vi "GOOP_ProviderClasses_SortingDialog.vi"(8 "error in (no error)":errorcluster) -> (0 "error out":errorcluster, 2 "Cancelled":bool, 3 "FirstProvider":string)   [LabVIEW 2020]
panel:
  in  "Cancel":bool
  in  "Save":bool
  in  "Down":bool
  in  "Up":bool
  in  "ClassProviders":i32(listbox) caption="Class Providers Order"
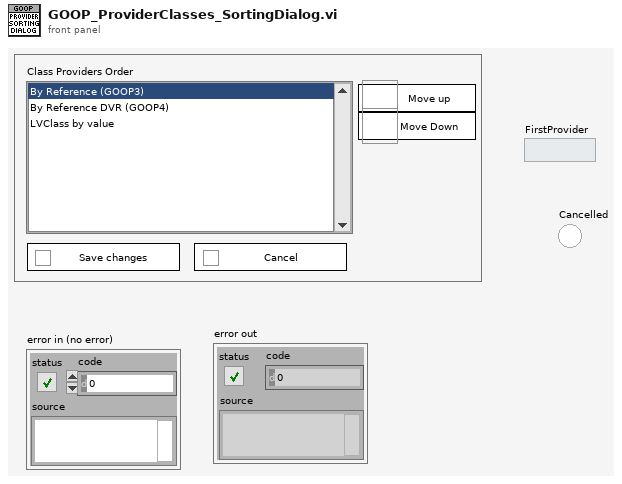
[diagram p1: front panel]
types:
  T1 = cluster{"Providers":cluster{"Provider":string, "Active":bool, "TranslatedName":string}[], "Provider":string, "Cancelled":bool}
  T2 = cluster{"Provider":string, "Active":bool, "TranslatedName":string}
  T3 = enum8{"Enabled", "Disabled", "Disabled and Grayed Out"}
  T4 = cluster{"Provider":string, "Active":bool, "TranslatedName":string}[]
  T5 = typedef "LVPoint32TypeDef.ctl" = cluster{"Horizontal":i32, "Vertical":i32}
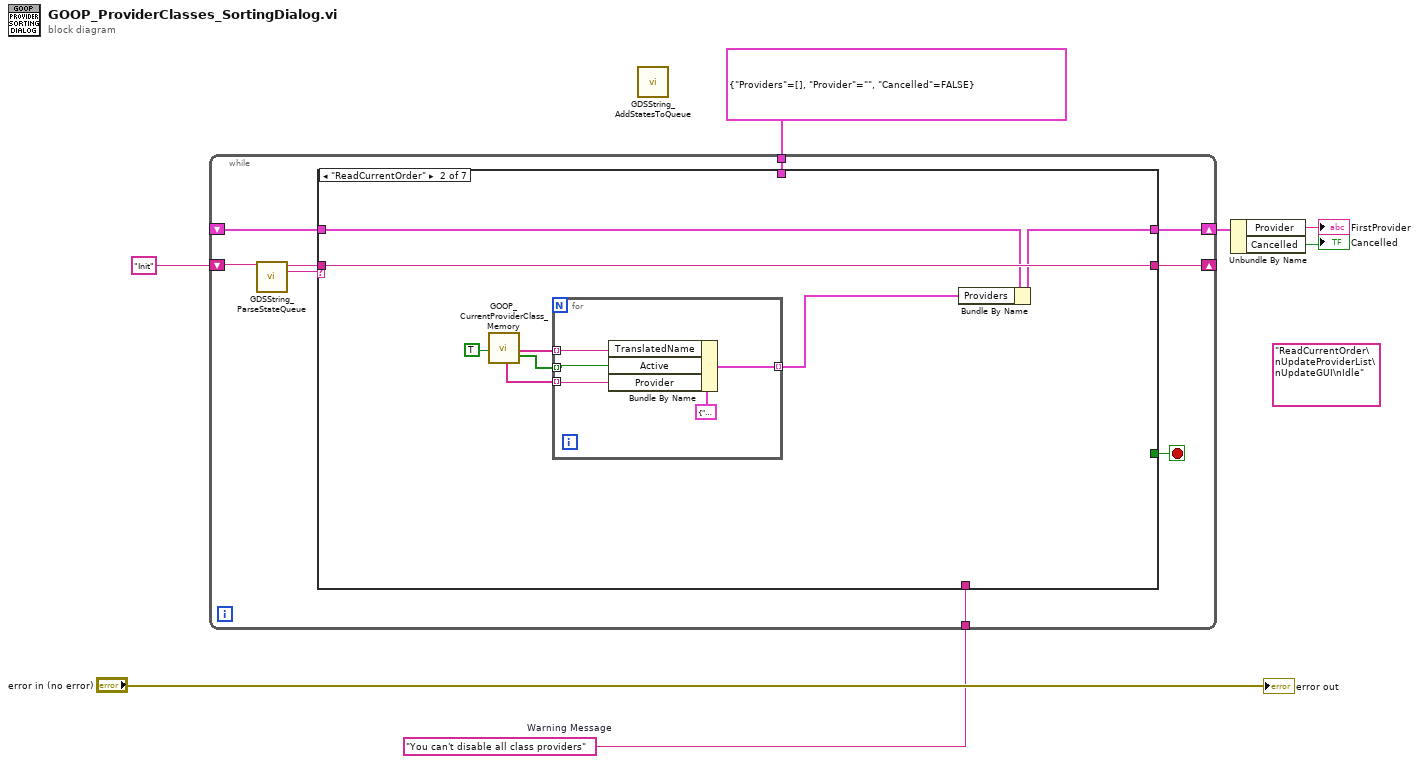
[diagram p0: block diagram]
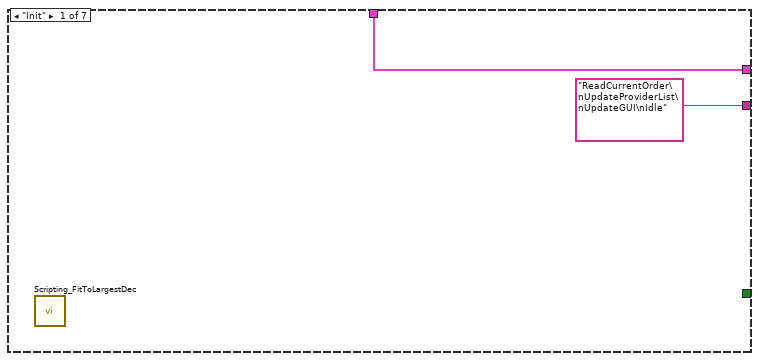
[diagram p2: hidden frame]
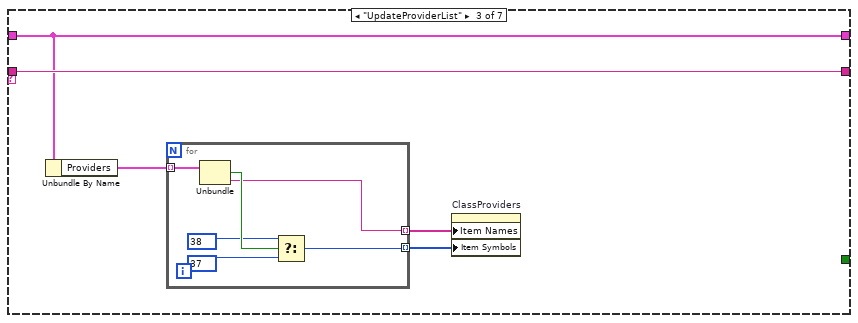
[diagram p3: hidden frame]
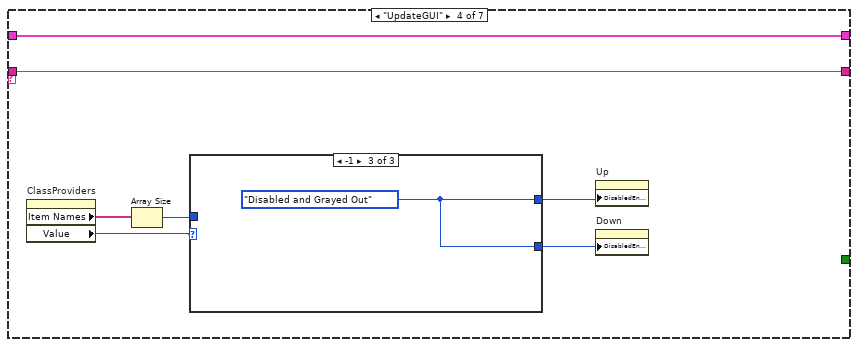
[diagram p4: hidden frame]
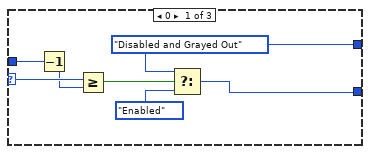
[diagram p5: hidden frame]
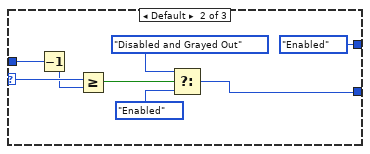
[diagram p6: hidden frame]
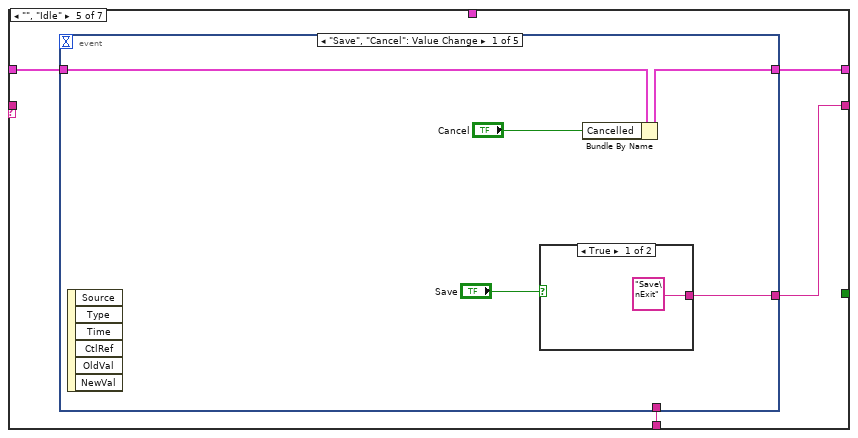
[diagram p7: hidden frame]
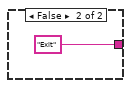
[diagram p8: hidden frame]
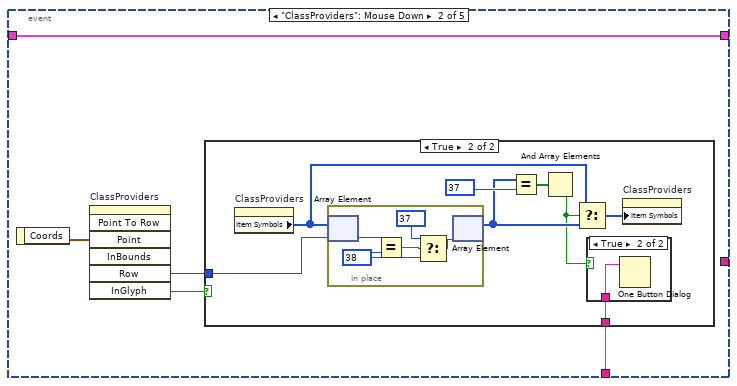
[diagram p9: hidden frame]
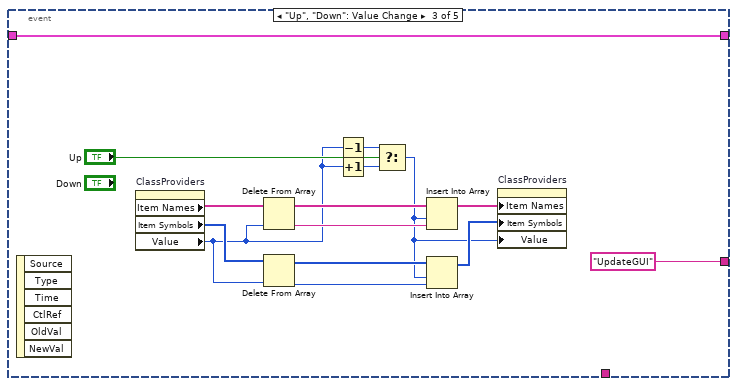
[diagram p12: hidden frame]
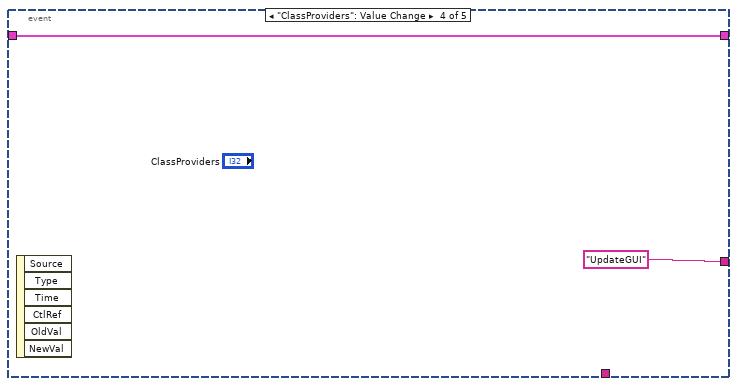
[diagram p13: hidden frame]
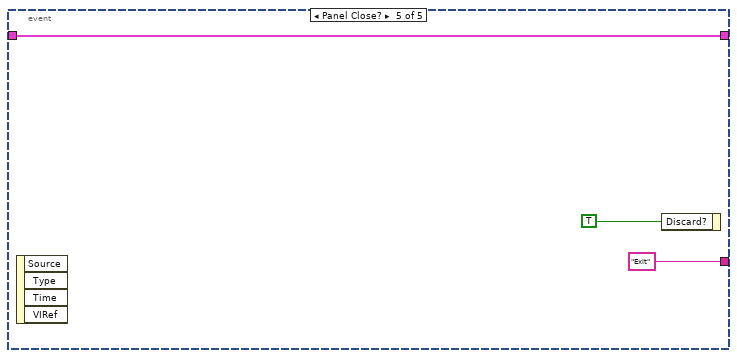
[diagram p14: hidden frame]
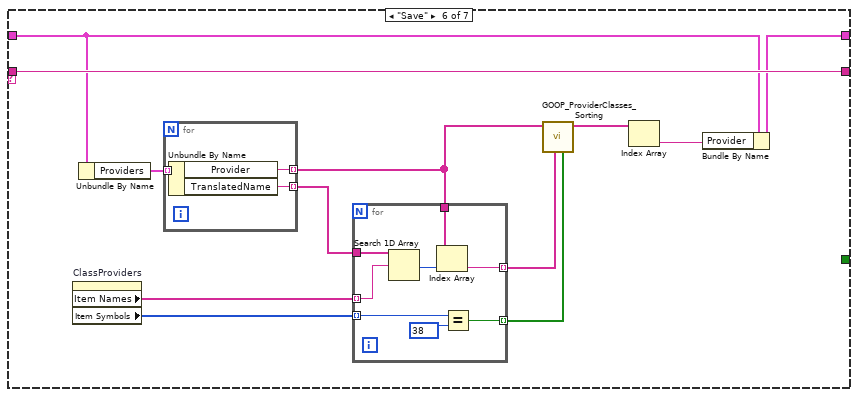
[diagram p15: hidden frame]
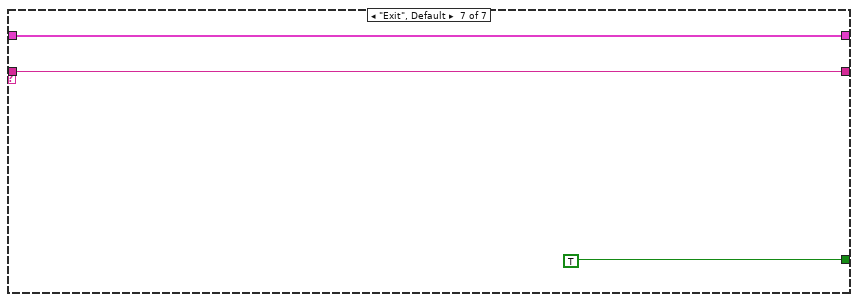
[diagram p16: hidden frame]
diagram:
  (unwired) "ReadCurrentOrder\nUpdateProviderList\nUpdateGUI\nIdle" ("Remaining States")
  w4 = "You can't disable all class providers"  # Warning Message
  n1 = while {
    shift-right: [w14] -> _
    shift-left: "Init" -> [w15]
    tunnel: T1 {"Providers"=[], "Provider"="", "Cancelled"=FALSE} -> [w11]
    shift-right: [w10] -> w3
    shift-left: _ -> [w9]
    tunnel: w4 -> [w8]
    stop <- w16 stop-if-true
    n2 = call "GDSString_ParseStateQueue.vi"("State Queue"=w15) -> ("Remaining States"=w12:string, "Current State"=w13:string)  [unwired: 10 in, 3 out]
    n3 = case shown="\"ReadCurrentOrder\"" w13 {
      tunnel: [_ _ _ _ _ _ TRUE] -> w16
      tunnel: ["ReadCurrentOrder\nUpdateProviderList\nUpdateGUI\nIdle" ("Remaining States") w26 w36 w49 w69 w127 w140] -> w14
      tunnel: w12 -> [_ w26 w36 w49 _ w127 w140]
      tunnel: [w18 w24 w35 w48 w66 w118 w139] -> w10
      tunnel: w11 -> [w18 _ _ _ _ _ _]
      tunnel: w9 -> [_ w25 w35 w48 w67 w126 w139]
      tunnel: w8 -> [_ _ _ _ w68 _ _]
      frame "Init" {
        n4 = call "Scripting_FitToLargestDec.vi"() -> ()  [unwired: 6 in, 2 out]
      }
      frame "ReadCurrentOrder" {
        n5 = call "GOOP_CurrentProviderClass_Memory.vi"("IgnoreFilter(False)"=TRUE) -> ("AllClassProviders(OriginalNames)"=w22:string[], "AllClassProviders(TranslatedNames)"=w21:string[], "AllClassProvidersFilterSettings"=w20:bool[])  [unwired: 12 in, 4 out]
        n6 = for {
          tunnel: w22 -> [w28] mode=indexing
          tunnel: w21 -> [w30] mode=indexing
          tunnel: w20 -> [w29] mode=indexing
          tunnel: [w27] -> w19 mode=indexing
          n7 = Bundle By Name(cluster=T2 {"Provider"="", "Active"=FALSE, "TranslatedName"=""} ("Cluster"), "TranslatedName"=w30, "Active"=w29, "Provider"=w28) -> (w27:T2)
        }
        n8 = Bundle By Name(cluster=w25, "Providers"=w19) -> (w24:T1)
      }
      frame "UpdateProviderList" {
        n9 = Unbundle By Name(w35) -> ("Providers"=w34:T4)
        n10 = for {
          tunnel: w34 -> [w42] mode=indexing
          tunnel: [w38] -> w32 mode=indexing
          tunnel: [w37] -> w33 mode=indexing
          n11 = Unbundle(w42) -> ("Active"=w41:bool, "TranslatedName"=w37:string)  [unwired: 1 out]
          n12 = Select(t=38, s=w41, f=37) -> (s? t:f=w38:i32)
        }
        n13 = property on="ClassProviders" class="LstBox (strict)"("Item Names"=w33, "Item Symbols"=w32) -> ()  [unwired: 2 in, 2 out]
      }
      frame "UpdateGUI" {
        n14 = property on="ClassProviders" class="LstBox (strict)"() -> ("Item Names"=w44:string[], "Value"=w47:i32)  [unwired: 2 in, 2 out]
        n15 = Array Size(array=w44) -> (size(s)=w43:i32)
        n16 = case shown="-1" w47 {
          selector: w47 -> [w56 w64 _]
          tunnel: [w51 T3."Enabled" ("Disabled") w65] -> w46
          tunnel: [w52 w60 w65] -> w45
          tunnel: w43 -> [w55 w63 _]
          frame 0 {
            w51 = T3."Disabled and Grayed Out" ("Disabled")
            n17 = Decrement(x=w55) -> (x-1=w54:i32)
            n18 = Greater Or Equal?(x=w56, y=w54) -> (x >= y?=w53:bool)
            n19 = Select(t=w51, s=w53, f=T3."Enabled" ("Disabled")) -> (s? t:f=w52:T3)
          }
          frame Default {
            n20 = Decrement(x=w63) -> (x-1=w62:i32)
            n21 = Greater Or Equal?(x=w64, y=w62) -> (x >= y?=w61:bool)
            n22 = Select(t=T3."Disabled and Grayed Out" ("Disabled"), s=w61, f=T3."Enabled" ("Disabled")) -> (s? t:f=w60:T3)
          }
          frame -1 {
            w65 = T3."Disabled and Grayed Out" ("Disabled")
          }
        }
        n23 = property on="Up" class="Bool"("DisabledEnum"=w46) -> ()  [unwired: 2 in, 2 out]
        n24 = property on="Down" class="Bool"("DisabledEnum"=w45) -> ()  [unwired: 2 in, 2 out]
      }
      frame "", "Idle" {
        n25 = event shown="[0] \"Save\", \"Cancel\": Value Change" {
          selector: _ -> [_ _ _ _ _]
          dyn-events: _ -> [_ _ _ _ _]
          timeout: _ -> [_ _ _ _ _]
          tunnel: [w74 _ "UpdateGUI" "UpdateGUI" "Exit"] -> w69
          tunnel: w68 -> [_ w78 _ _ _]
          tunnel: w67 -> [w72 w77 w96 w111 w113]
          tunnel: [w71 w77 w96 w111 w113] -> w66
          event "Save", "Cancel": Value Change {
            n26 = event-data() -> ()  [unwired: 1 in, 6 out]
            n27 = case shown="True" "Save" {
              tunnel: ["Save\nExit" "Exit"] -> w74
              frame True {
              }
              frame False {
              }
            }
            n28 = Bundle By Name(cluster=w72, "Cancelled"="Cancel") -> (w71:T1)
          }
          event "ClassProviders": Mouse Down {
            n29 = event-data() -> ("Coords"=w81:T5)  [unwired: 1 in]
            n30 = invoke on="ClassProviders" class="LstBox (strict)" method="Point To Row"("Point"=w81) -> ("Row"=w79:i32, "InGlyph"=w80:bool)  [unwired: 6 in, 5 out]
            n31 = case shown="True" w80 {
              tunnel: w79 -> [_ w89]
              tunnel: w78 -> [_ w82]
              frame False {
              }
              frame True {
                n32 = property on="ClassProviders" class="LstBox (strict)"() -> ("Item Symbols"=w85:i32[])  [unwired: 2 in, 2 out]
                n33 = in-place {
                  w93 = 38
                  n34 = in-place-array #1(w85, w89) -> (w95:i32)
                  n35 = Equal?(x=w95, y=w93) -> (x = y?=w94:bool)
                  n36 = Select(t=37, s=w94, f=w93) -> (s? t:f=w91:i32)
                  n37 = in-place-array #1(w91) -> (w86:i32[])  [unwired: 1 out]
                }
                n38 = Equal?(x=w86, y=37) -> (x = y?=w87:bool[])
                n39 = And Array Elements(Boolean array=w87) -> (logical AND=w83:bool)
                n40 = Select(t=w85, s=w83, f=w86) -> (s? t:f=w84:i32[])
                n41 = case shown="True" w83 {
                  tunnel: w82 -> [_ w90]
                  frame False {
                  }
                  frame True {
                    n42 = One Button Dialog(message=w90) -> ()  [unwired: 1 in, 1 out]
                  }
                }
                n43 = property on="ClassProviders" class="LstBox (strict)"("Item Symbols"=w84) -> ()  [unwired: 2 in, 2 out]
              }
            }
          }
          event "Up", "Down": Value Change {
            n44 = event-data() -> ()  [unwired: 1 in, 6 out]
            n45 = property on="ClassProviders" class="LstBox (strict)"() -> ("Item Names"=w109:string[], "Item Symbols"=w108:i32[], "Value"=w99:i32)  [unwired: 2 in, 2 out]
            n46 = Delete From Array(array=w109, index=w99) -> (deleted portion=w105:string, array with subset deleted=w107:string[])  [unwired: 1 in]
            n47 = Delete From Array(array=w108, index=w99) -> (deleted portion=w104:i32, array with subset deleted=w106:i32[])  [unwired: 1 in]
            n48 = Decrement(x=w99) -> (x-1=w98:i32)
            n49 = Increment(x=w99) -> (x+1=w97:i32)
            n50 = Select(t=w98, s="Up", f=w97) -> (s? t:f=w100:i32)
            n51 = Insert Into Array(array=w107, index=w100, new element=w105) -> (w102:string[])
            n52 = Insert Into Array(array=w106, index=w100, new element=w104) -> (w101:i32[])
            n53 = property on="ClassProviders" class="LstBox (strict)"("Item Names"=w102, "Item Symbols"=w101, "Value"=w100) -> ()  [unwired: 2 in, 2 out]
          }
          event "ClassProviders": Value Change {
            n54 = event-data() -> ()  [unwired: 1 in, 6 out]
          }
          event Panel Close? {
            n55 = event-data() -> ()  [unwired: 1 in, 4 out]
            n56 = event-data("Discard?"=TRUE) -> ()  [unwired: 1 in, 1 out]
          }
        }
      }
      frame "Save" {
        n57 = property on="ClassProviders" class="LstBox (strict)"() -> ("Item Names"=w123:string[], "Item Symbols"=w121:i32[])  [unwired: 2 in, 2 out]
        n58 = Unbundle By Name(w126) -> ("Providers"=w125:T4)
        n59 = for {
          tunnel: w125 -> [w138] mode=indexing
          tunnel: [w137] -> w116 mode=indexing
          tunnel: [w136] -> w124 mode=indexing
          n60 = Unbundle By Name(w138) -> ("Provider"=w137:string, "TranslatedName"=w136:string)
        }
        n61 = for {
          tunnel: w124 -> [w135]
          tunnel: w123 -> [w134] mode=indexing
          tunnel: w116 -> [w133]
          tunnel: [w131] -> w122 mode=indexing
          tunnel: w121 -> [w130] mode=indexing
          tunnel: [w128] -> w120 mode=indexing
          n62 = Search 1D Array(1D array=w135, element=w134) -> (index of element=w132:i32)  [unwired: 1 in]
          n63 = Index Array(array=w133, index=w132) -> (element=w131:string)
          n64 = Equal?(x=w130, y=38) -> (x = y?=w128:bool)
        }
        n65 = call "GOOP_ProviderClasses_Sorting.vi"("ProvidersClassesActive"=w120, "ProvidersClassesSortOrder"=w122, "AllClassProvidersIn(OriginalNames)"=w116) -> ("AllClassProvidersOut(OriginalNames)"=w119:string[])  [unwired: 6 in, 2 out]
        n66 = Index Array(array=w119) -> (element=w117:string)  [unwired: 1 in]
        n67 = Bundle By Name(cluster=w126, "Provider"=w117) -> (w118:T1)
      }
      frame "Exit", Default {
      }
    }
  }
  n68 = call "GDSString_AddStatesToQueue.vi"() -> ()  [unwired: 15 in, 1 out]
  n69 = Unbundle By Name(w3) -> ("Provider"=→"FirstProvider":string, "Cancelled"=→"Cancelled":bool)
  "error out" <- "error in (no error)"
